vi "Test Hide panel.vi"() -> ()   [LabVIEW 2012]
uses:
  Hide Panel.xctl
panel:
  out "Hide Panel":bool(xcontrol)
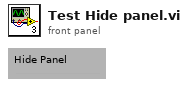
[diagram p1: front panel]
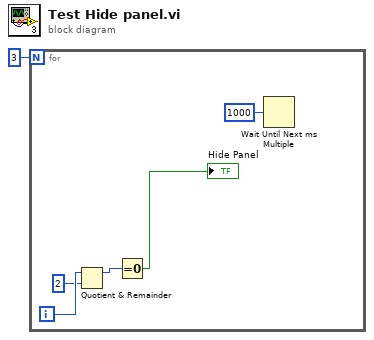
[diagram p0: block diagram]
diagram:
  n1 = for {
    N: 3 -> [_]
    i -> [w6]
    n2 = Quotient & Remainder(x=w6, y=2) -> (x-y*floor(x/y)=w4:i32)  [unwired: 1 out]
    n3 = Equal To 0?(x=w4) -> (x = 0?=→"Hide Panel":bool)
    n4 = Wait Until Next ms Multiple(millisecond multiple=u32 1000) -> ()  [unwired: 1 out]
  }
